vi "Write to DB as list.vi"(8 "error in (no error)":errorcluster, 11 "Database Entry in":refnum<class "Database Entry.lvclass">) -> (0 "error out":errorcluster, 2 "Stack names":string[](array[string]), 3 "Database Entry out":refnum<class "Database Entry.lvclass">)   [LabVIEW 2021, in "Database Entry.lvclass"]
uses:
  Database Entry.lvclass
  Database Entry.lvclass/Database Entry.ctl
  <vilib>/Utility/file.llb/Read Delimited Spreadsheet (string).vi
  <vilib>/Utility/file.llb/Write Delimited Spreadsheet (string).vi
  Components/Stack/Stack.lvclass
panel:
  out "Data cluster":T1={"module or proto"="proto", " geometry"="full", "resolution"="LD", "baselayer"="BA_123", "toplayer"="SI_789", "bl_pos"="1", "tl_pos"="1", "put_pos"="1", "region"="1", "asstray"="1", "comptray"="1", "put"="1", "date"="2024-04-02", "timestart"="1:12:12.442", "timeend"="1:23:45.244", "operator"="cmuperson", "tape"="some", "glue"="some", "stack name"="some", "Adhesive type"="", "Comments"="", "Temperature"="", "Relative Humidity"=""}
  out "error out py":errorcluster
  out "String Out":string="Upload Success"
  in  "error in (no error) py":errorcluster
  # "Debug instructions\n#### The order of values in db_data_cols must match the order of values in Data cluster in Stack.lvclass: Get stack data.vi \n#### The variable names below correspond to postgres col name. LV does not neet to match the col numes but just the values. \n#### Right-click on the Data cluster on the front panel and click on 'reorder controls' to verify the order is correct in the code. \n#### The physical position of the fields is different from the actual position.\n\nIn Main VIs/python_db/postgres_tools.py, see functions 'assembly_data' and 'assembly_data_as_list'."
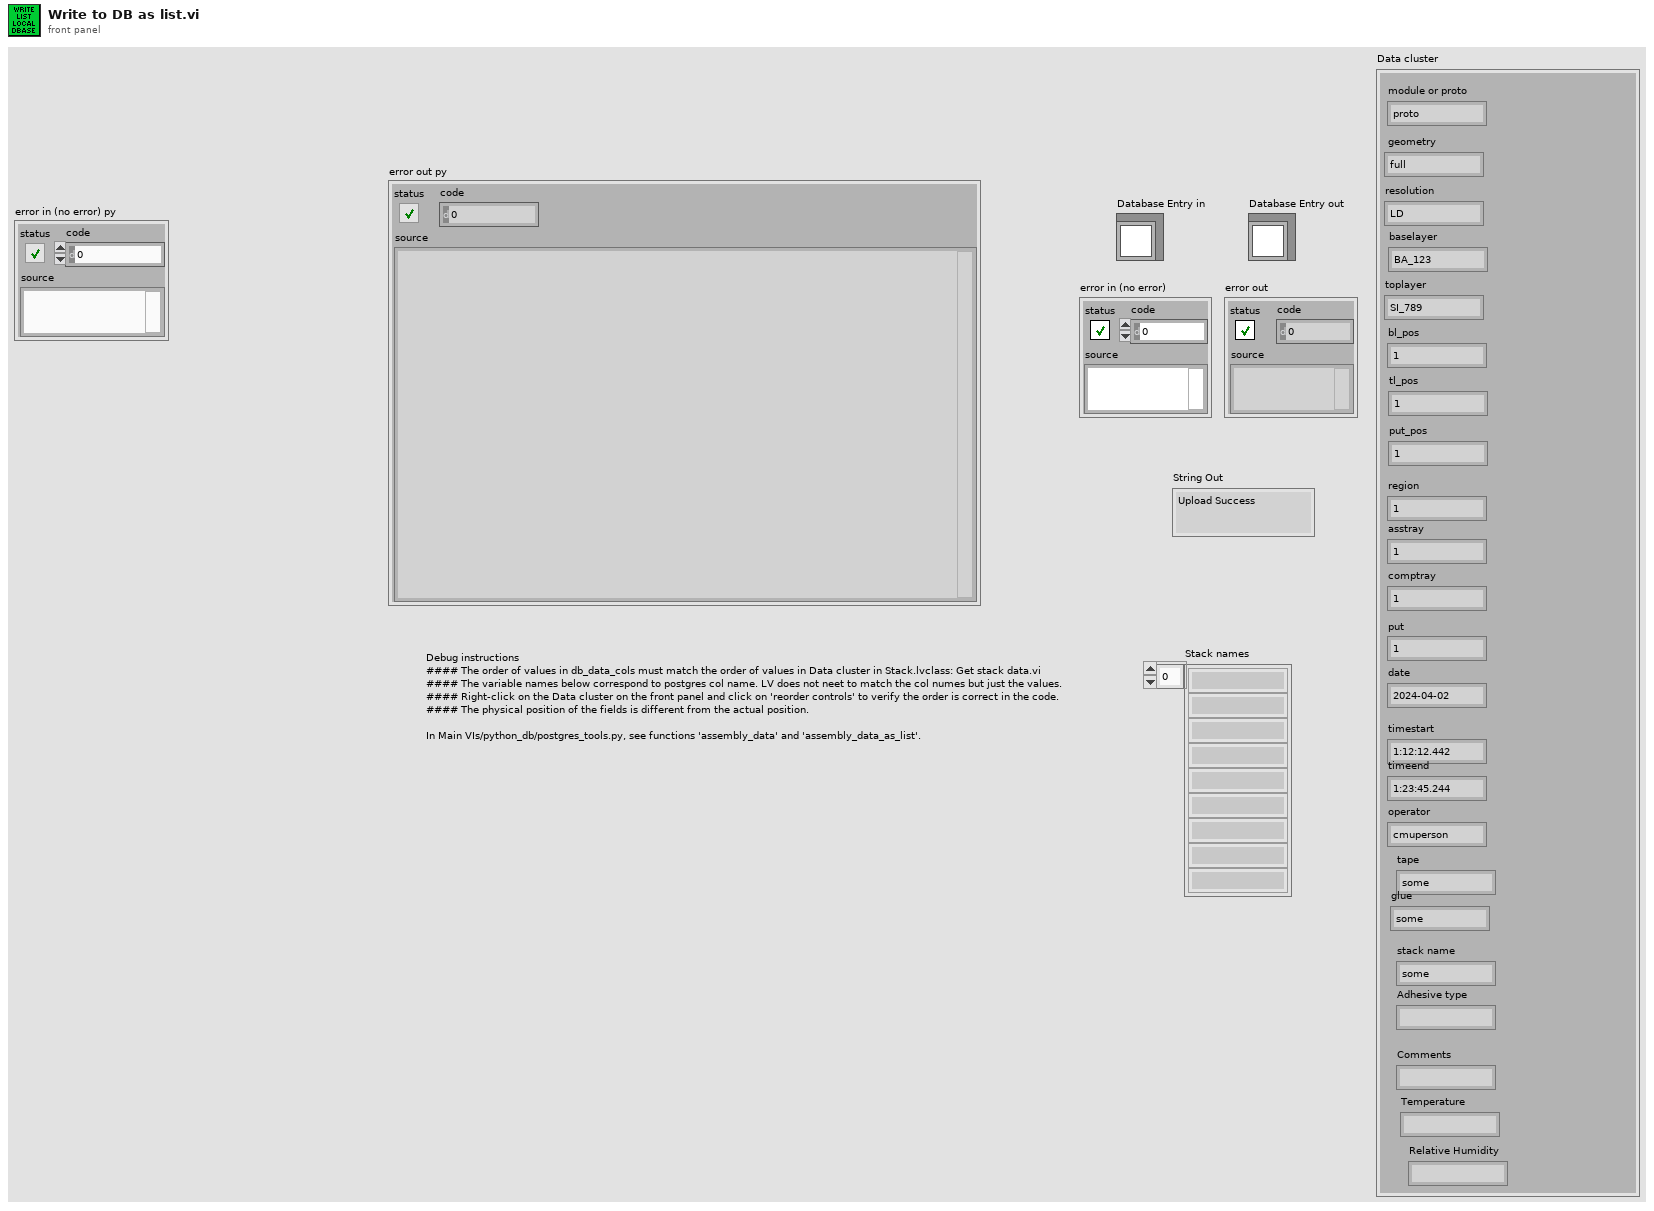
[diagram p1: front panel]
types:
  T1 = cluster{"module or proto":string, " geometry":string, "resolution":string, "baselayer":string, "toplayer":string, "bl_pos":string, "tl_pos":string, "put_pos":string, "region":string, "asstray":string, "comptray":string, "put":string, "date":string, "timestart":string, "timeend":string, "operator":string, "tape":string, "glue":string, "stack name":string, "Adhesive type":string, "Comments":string, "Temperature":string, "Relative Humidity":string}
  T2 = typedef "File Paths.ctl" = cluster{"Glue Pattern Folder":path, "Carrier Tray Folder":path, "Pick Up Tool Fixture Folder":path, "Components Folder":path, "Bellows Tool Offset.txt":path, "Pick Up Tool Offset.txt":path, "Dispense Tip Offset.txt":path, "Log Files":path, "Gantry Assembly Map.txt":path, "Syringe and offset map.txt":path, "Controllers Folder":path, "Local dbase config":path}
  T3 = cluster{"type (proto/module)":string, " geometry":string, "resolution":string, "baselayer":string, "toplayer":string, "bl_pos":string, "tl_pos":string, "put_pos":string, "region":string, "asstray":string, "comptray":string, "put":string, "date":string, "timestart":string, "timeend":string, "operator":string, "tape":string, "glue":string, "stack name":string, "Adhesive type":string, "Comments":string, "Temperature":string, "Relative Humidity":string}
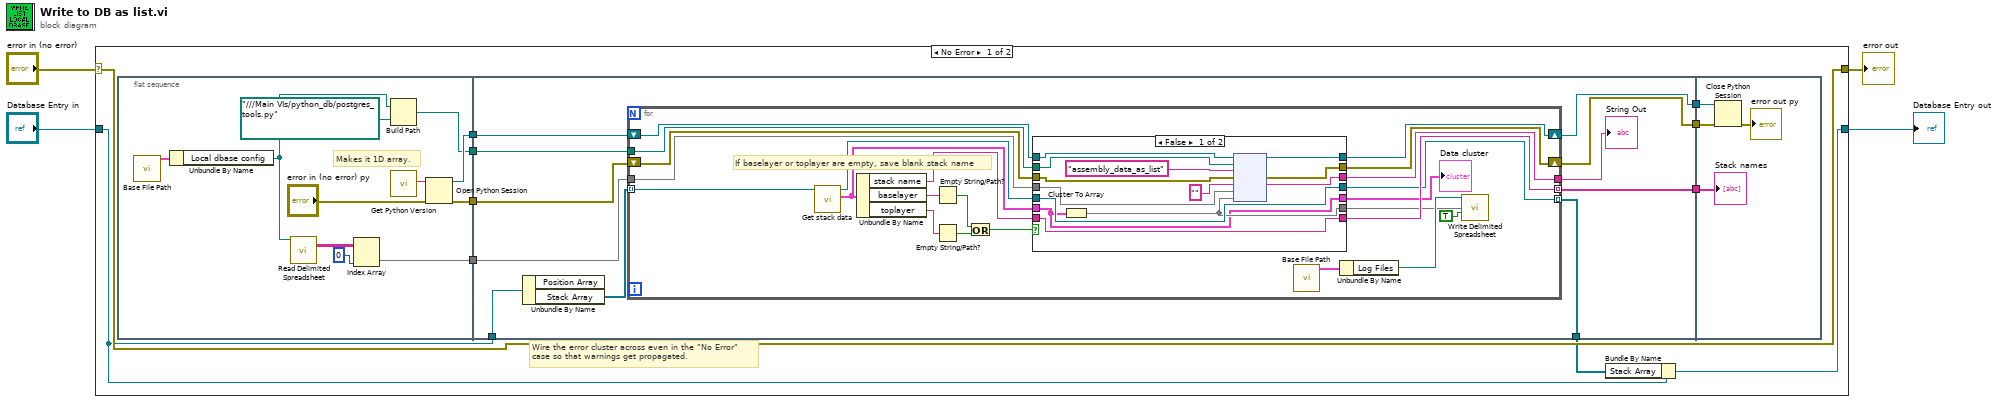
[diagram p0: block diagram]
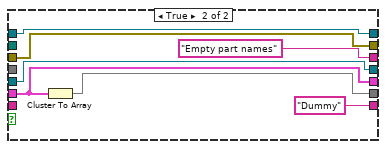
[diagram p2: hidden frame]
diagram:
  n1 = case shown="No Error" "error in (no error)" {
    selector: "error in (no error)" -> [w15 w86]
    tunnel: [w15 w86] -> w3
    tunnel: [w7 w85] -> w1
    tunnel: "Database Entry in" -> [w6 w85]
    frame No Error {
      # "Wire the error cluster across even in the \"No Error\"\ncase so that warnings get propagated."
      n2 = flat-sequence {
        tunnel: [w25] -> w14
        tunnel: [w26] -> w13
        tunnel: [w22] -> w12
        tunnel: [w18] -> w11
        tunnel: [w36] -> w10
        tunnel: [w35] -> w9
        tunnel: w14 -> [w37]
        tunnel: w13 -> [w34]
        tunnel: w12 -> [w33]
        tunnel: w11 -> [w32]
        tunnel: w6 -> [w31]
        tunnel: [w28] -> w8
        tunnel: [w27] -> w5
        tunnel: w10 -> [w83]
        tunnel: w9 -> [w84]
        tunnel: w8 -> [w81]
        frame #0 {
          # "Makes it 1D array."
          n3 = call "Base File Path.vi"() -> ("Paths Out"=w23:T2)  [unwired: 11 in]
          n4 = Unbundle By Name(w23) -> ("Local dbase config"=w21:path)
          n5 = call-poly <vilib>:"Read Delimited Spreadsheet.vi"("file path (dialog if empty)"=w21) -> ("all rows"=w20:string[][])  [unwired: 9 in, 5 out]
          n6 = Index Array(array=w20, index (col)=0 ("disabled index (col)")) -> (element=w18:string[])  [unwired: 1 in]
          n7 = Build Path(base path=w21, name or relative path=path "../../../Main VIs/python_db/postgres_tools.py" ("module path")) -> (appended path=w22:path)
          n8 = call "Get Python Version.vi"() -> ("Python Version"=w16:string)  [unwired: 10 in, 1 out]
          n9 = Open Python Session(python version=w16, 3:"error in (no error) py") -> (session out=w26:refnum<k35>, error out=w25:errorcluster)  [unwired: 1 in]
        }
        frame #1 {
          n10 = Unbundle By Name(w31) -> ("Stack Array"=w29:refnum<class "Stack.lvclass">[])  [unwired: 1 out]
          n11 = for {
            tunnel: w33 -> [w52]
            shift-right: [w60] -> w36
            shift-left: w37 -> [w51]
            shift-right: [w59] -> w35
            shift-left: w34 -> [w53]
            tunnel: [w58] -> w30
            tunnel: w29 -> [w57] mode=indexing
            tunnel: w32 -> [w54]
            tunnel: [w48] -> w28 mode=indexing
            tunnel: [w39] -> w27 mode=indexing
            # "If baselayer or toplayer are empty, save blank stack name"
            n12 = call "Get stack data.vi"("Stack in"=w57) -> ("Data cluster"=w45:T3, "Stack out"=w44:refnum<class "Stack.lvclass">)  [unwired: 8 in, 1 out]
            n13 = Unbundle By Name(w45) -> ("stack name"=w43:string, "baselayer"=w42:string, "toplayer"=w41:string)
            n14 = Empty String/Path?(string/path=w42) -> (empty?=w50:bool)
            n15 = Empty String/Path?(string/path=w41) -> (empty?=w49:bool)
            n16 = Or(x=w50, y=w49) -> (x .or. y?=w47:bool)
            n17 = case shown="False" w47 {
              tunnel: [w73 w79] -> w60
              tunnel: [w72 w80] -> w59
              tunnel: [w71 "Empty part names"] -> w58
              tunnel: w54 -> [w69 _]
              tunnel: w53 -> [w68 w80]
              tunnel: w52 -> [w67 _]
              tunnel: w51 -> [w66 w79]
              tunnel: w43 -> [w64 _]
              tunnel: [w64 "Dummy" ("stack name")] -> w48
              tunnel: w45 -> [w61 w74]
              tunnel: [w62 w75] -> w40
              tunnel: w44 -> [w63 w76]
              tunnel: [w63 w76] -> w39
              tunnel: [w61 w74] -> w38
              frame False {
                n18 = Cluster To Array(cluster=w61) -> (array=w62:string[])
                n19 = node(w68, w67, "assembly_data_as_list" ("function name"), w66, "", w69, w62) -> (w72:refnum<k35>, w73:errorcluster, w71:string)  [unwired: 2 in, 2 out]
              }
              frame True {
                n20 = Cluster To Array(cluster=w74) -> (array=w75:string[])
              }
            }
            "Data cluster" <- w38
            n21 = call "Base File Path.vi"() -> ("Paths Out"=w56:T2)  [unwired: 11 in]
            n22 = Unbundle By Name(w56) -> ("Log Files"=w55:path)
            n23 = call-poly <vilib>:"Write Delimited Spreadsheet.vi"("file path (dialog if empty)"=w55, "1D data"=w40, "append to file? (new file:F)"=TRUE) -> ()  [unwired: 11 in, 2 out]
          }
          "String Out" <- w30
        }
        frame #2 {
          n24 = Close Python Session(session in=w84, error in=w83) -> (11:→"error out py":errorcluster)
          "Stack names" <- w81
        }
      }
      n25 = Bundle By Name(cluster=w6, "Stack Array"=w5) -> (w7:refnum<class "Database Entry.lvclass">)
    }
    frame Error {
    }
  }
  "error out" <- w3
  "Database Entry out" <- w1
